vi "Native_GetPanelControls.vi"() -> ()   [LabVIEW 2024]
panel:
  out "error out":errorcluster caption="错误输出"
  out "control_ids":u32[](array[numeric])
  in  "control_ids type":u32
  in  "target_path":path
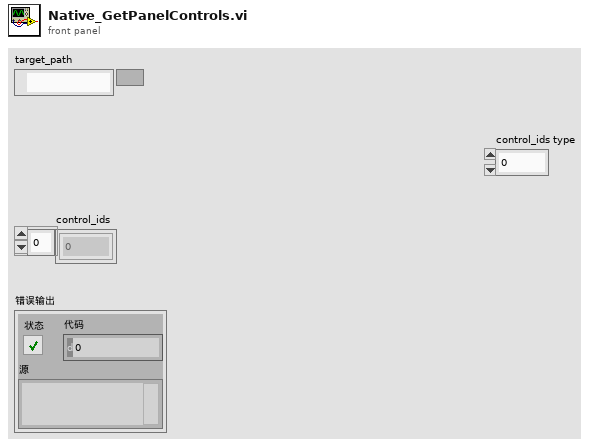
[diagram p1: front panel]
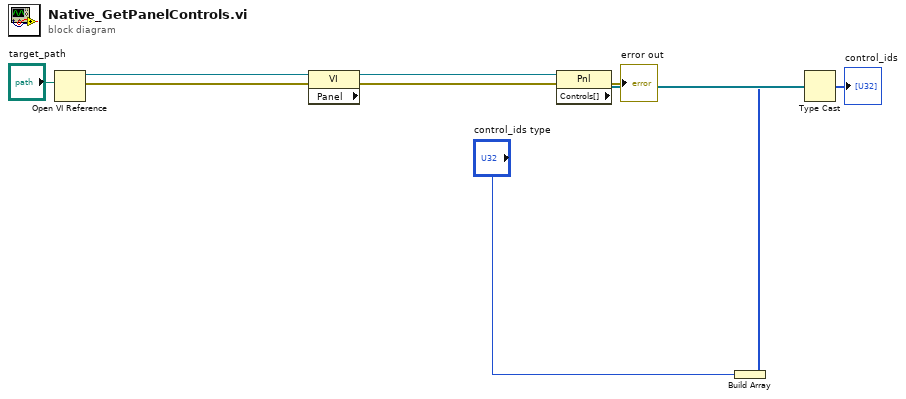
[diagram p0: block diagram]
diagram:
  n1 = Open VI Reference ("打开VI引用")(vi path="target_path") -> (vi reference=w9:refnum<vi>, error out=w8:errorcluster)  [unwired: 5 in]
  n2 = property on="属性节点" class="VI"(reference=w9, error in=w8) -> (error out=w6:errorcluster, "Panel"=w7:refnum<vi>)  [unwired: 1 out]
  n3 = property on="属性节点" class="Pnl"(reference=w7, error in=w6) -> (error out=→"error out":errorcluster, "Controls[]"=w5:refnum<vi>[])  [unwired: 1 out]
  n4 = Build Array ("创建数组")("control_ids type") -> (w3:u32[])
  n5 = Type Cast ("强制类型转换")(type=w3, x=w5) -> (*(type *) &x=→"control_ids":u32[])
